vi "Load_Rabi_MW_Change.vi"(0 "Numeric 2":i32, 1 "Numeric":i32, 2 "?":bool=TRUE, 3 "MW Step Size":dbl=2e-09) -> (7 "MW":dbl)   [LabVIEW 2024]
uses:
  <vilib>/Utility/error.llb/DialogTypeEnum.ctl
  SpinCore_API_file_location.vi
panel:
  out "x+y 3":dbl
  out "output array 2":T1(array[cluster])
  out "x+y 2":dbl
  out "output array":T1(array[cluster])
  in  "Instructions":T1(array[cluster])=[{"Instruct Data"=0, "Op Code"=0, "Flags"=[FALSE, FALSE, TRUE, FALSE, FALSE, FALSE, FALSE, TRUE, FALSE, FALSE, FALSE, FALSE, FALSE, FALSE, FALSE, FALSE, FALSE, FALSE, FALSE, FALSE, FALSE, FALSE, FALSE, TRUE], "Comments"="0 Dark", "Time (s)"=6e-06}, {"Instruct Data"=0, "Op Code"=0, "Flags"=[TRUE, FALSE, FALSE, FALSE, TRUE, FALSE, FALSE, TRUE, FALSE, FALSE, FALSE, FALSE, FALSE, FALSE, FALSE, FALSE, FALSE, FALSE, FALSE, FALSE, FALSE, FALSE, FALSE, FALSE], "Comments"="1 PI", "Time (s)"=1e-08}, {"Instruct Data"=0, "Op Code"=0, "Flags"=[FALSE, TRUE, FALSE, FALSE, FALSE, FALSE, FALSE, TRUE, FALSE, FALSE, FALSE, FALSE, FALSE, FALSE, FALSE, FALSE, FALSE, FALSE, FALSE, FALSE, FALSE, FALSE, FALSE, FALSE], "Comments"="2 AOM Delay", "Time (s)"=5e-07}, {"Instruct Data"=0, "Op Code"=0, "Flags"=[FALSE, TRUE, FALSE, FALSE, FALSE, FALSE, FALSE, FALSE, FALSE, FALSE, FALSE, FALSE, FALSE, FALSE, FALSE, FALSE, FALSE, FALSE, FALSE, FALSE, FALSE, FALSE, FALSE, FALSE], "Comments"="3 AOM inhibit off", "Time (s)"=5e-07}, {"Instruct Data"=0, "Op Code"=0, "Flags"=[FALSE, TRUE, FALSE, FALSE, FALSE, FALSE, FALSE, TRUE, FALSE, FALSE, FALSE, FALSE, FALSE, FALSE, FALSE, FALSE, FALSE, FALSE, FALSE, FALSE, FALSE, FALSE, FALSE, FALSE], "Comments"="4 AOM", "Time (s)"=5e-06}, {"Instruct Data"=0, "Op Code"=0, "Flags"=[FALSE, FALSE, FALSE, FALSE, FALSE, FALSE, FALSE, TRUE, FALSE, FALSE, FALSE, FALSE, FALSE, FALSE, FALSE, FALSE, FALSE, FALSE, FALSE, FALSE, FALSE, FALSE, FALSE, FALSE], "Comments"="5 Dark", "Time (s)"=6e-06}, {"Instruct Data"=0, "Op Code"=0, "Flags"=[FALSE, TRUE, FALSE, FALSE, FALSE, FALSE, FALSE, TRUE, FALSE, FALSE, FALSE, FALSE, FALSE, FALSE, FALSE, FALSE, FALSE, FALSE, FALSE, FALSE, FALSE, FALSE, FALSE, FALSE], "Comments"="6 AOM delay", "Time (s)"=5e-07}, {"Instruct Data"=0, "Op Code"=0, "Flags"=[FALSE, TRUE, FALSE, FALSE, FALSE, FALSE, FALSE, FALSE, FALSE, FALSE, FALSE, FALSE, FALSE, FALSE, FALSE, FALSE, FALSE, FALSE, FALSE, FALSE, FALSE, FALSE, FALSE, FALSE], "Comments"="7 AOM inhibit", "Time (s)"=5e-07}, {"Instruct Data"=0, "Op Code"=6, "Flags"=[FALSE, TRUE, FALSE, FALSE, FALSE, FALSE, FALSE, TRUE, FALSE, FALSE, FALSE, FALSE, FALSE, FALSE, FALSE, FALSE, FALSE, FALSE, FALSE, FALSE, FALSE, FALSE, FALSE, FALSE], "Comments"="8 AOM", "Time (s)"=5e-06}, {"Instruct Data"=0, "Op Code"=0, "Flags"=[FALSE, TRUE, FALSE, FALSE, FALSE, FALSE, FALSE, FALSE, FALSE, FALSE, FALSE, FALSE, FALSE, FALSE, FALSE, FALSE, FALSE, FALSE, FALSE, FALSE, FALSE, FALSE, FALSE, FALSE], "Comments"="9", "Time (s)"=2e-06}, {"Instruct Data"=0, "Op Code"=0, "Flags"=[FALSE, TRUE, TRUE, FALSE, FALSE, FALSE, FALSE, FALSE, FALSE, FALSE, FALSE, FALSE, FALSE, FALSE, FALSE, FALSE, FALSE, FALSE, FALSE, FALSE, FALSE, FALSE, FALSE, FALSE], "Comments"="10", "Time (s)"=1e-07}, {"Instruct Data"=0, "Op Code"=0, "Flags"=[FALSE, TRUE, FALSE, FALSE, FALSE, FALSE, FALSE, FALSE, FALSE, FALSE, FALSE, FALSE, FALSE, FALSE, FALSE, FALSE, FALSE, FALSE, FALSE, FALSE, FALSE, FALSE, FALSE, FALSE], "Comments"="11", "Time (s)"=2.9e-06}, {"Instruct Data"=0, "Op Code"=6, "Flags"=[FALSE, FALSE, FALSE, FALSE, FALSE, FALSE, FALSE, FALSE, FALSE, FALSE, FALSE, FALSE, FALSE, FALSE, FALSE, FALSE, FALSE, FALSE, FALSE, FALSE, FALSE, FALSE, FALSE, FALSE], "Comments"="12", "Time (s)"=1e-06}] {"Time (s)" format="%.3p"; "Op Code" items=["Continue", "Stop", "Loop", "End Loop", "JSR", "RTS", "Branch", "Long Delay", "Wait"]}
  in  "# of Instructions":u32=9
  in  "clock_freq (MHz)":dbl=500.0
  # "1) MW indicator\n2) AOM\n3) DAQ\n4) I\n5)Q\n8) Inhibit\n24) Start_Trig"
  # "1"
  # "2"
  # "3"
  # "4"
  # "5"
  # "6"
  # "7"
  # "8"
  # "9"
  # "10"
  # "11"
  # "12"
  # "13"
  # "14"
  # "15"
  # "16"
  # "17"
  # "18"
  # "19"
  # "20"
  # "21"
  # "22"
  # "23"
  # "24"
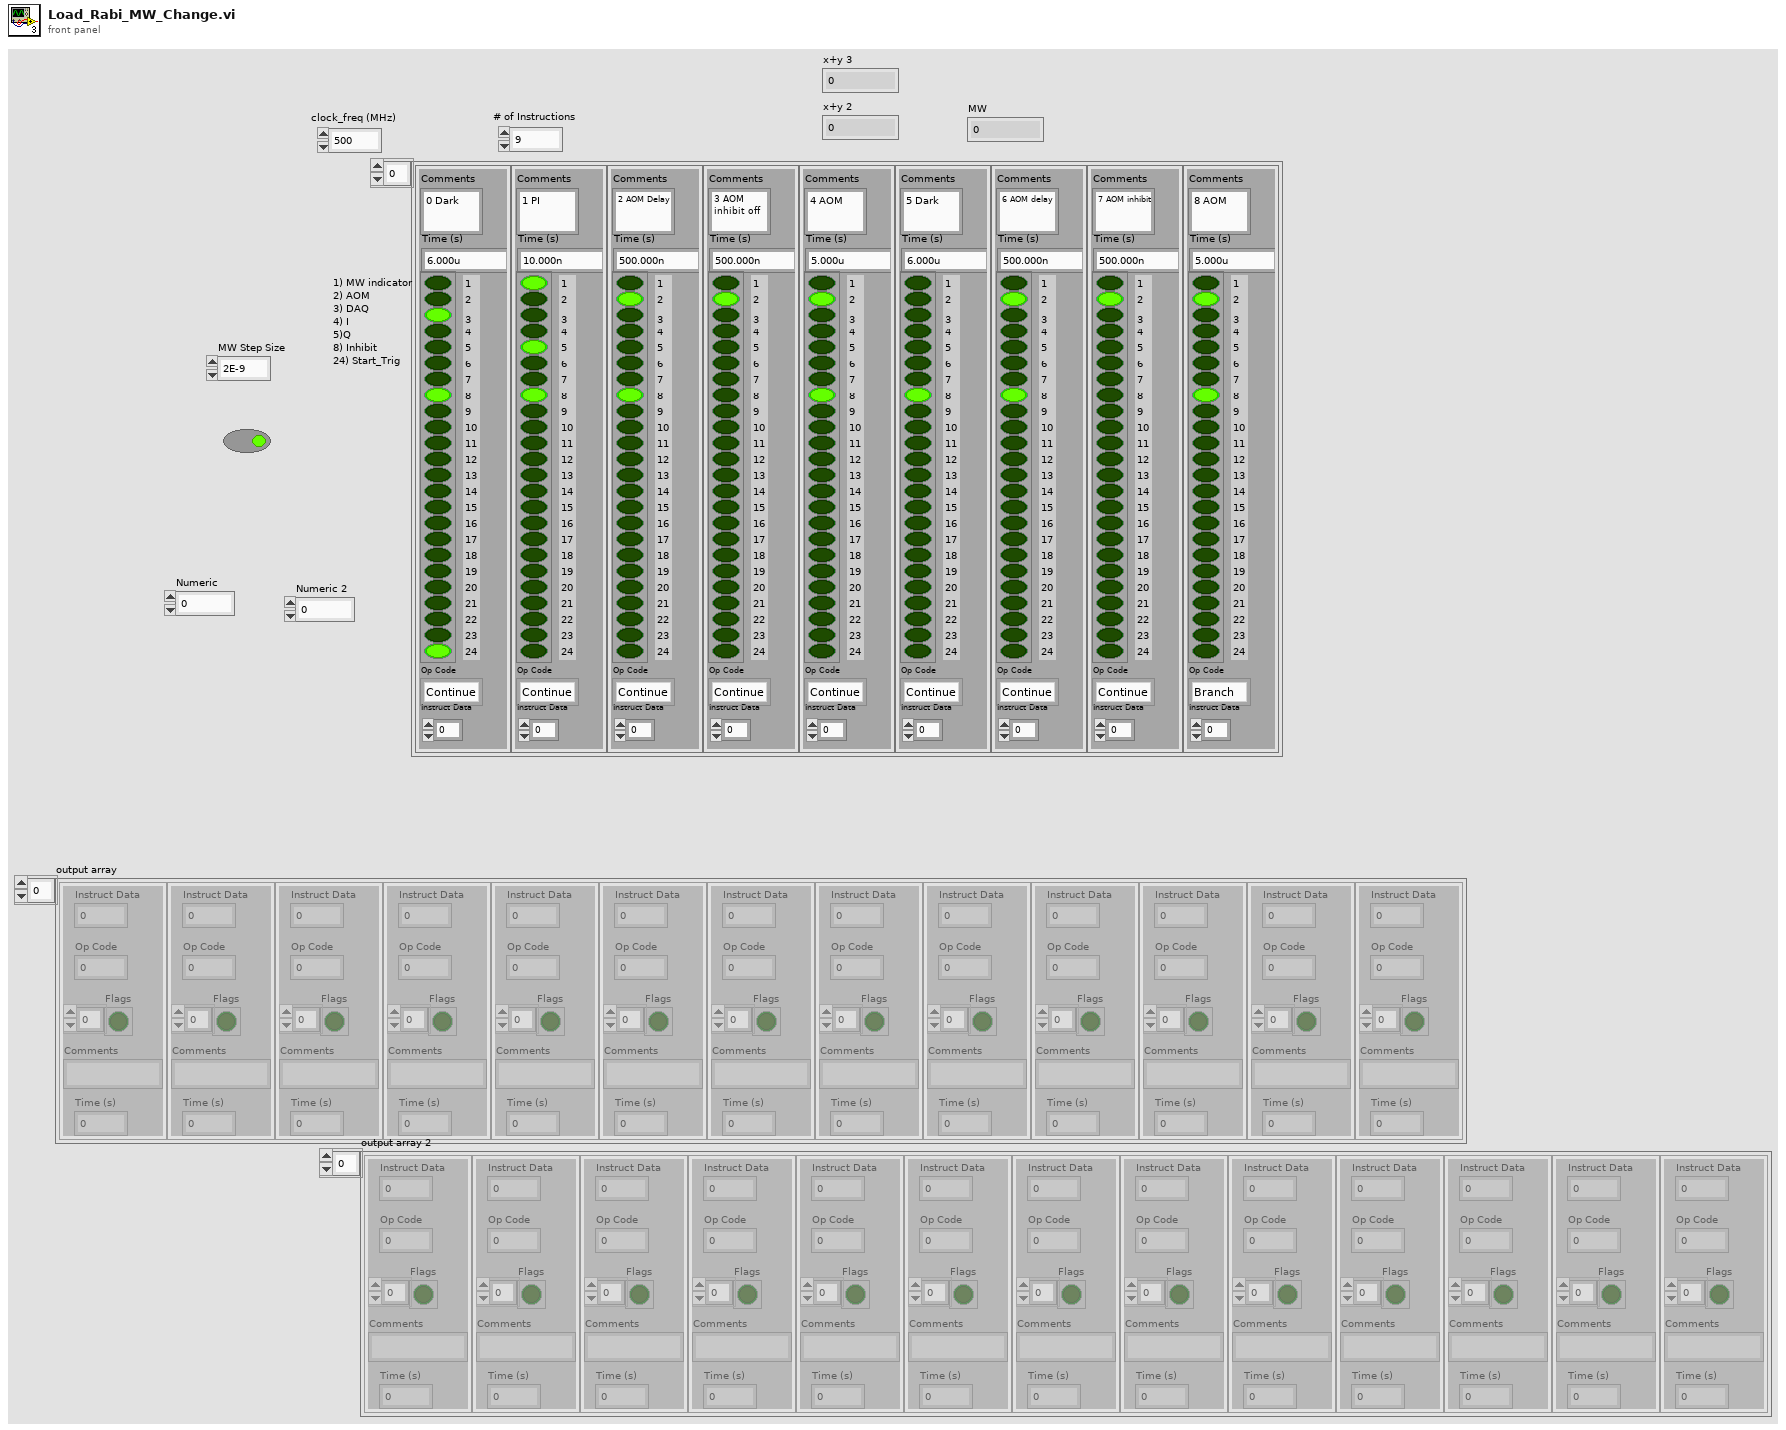
[diagram p1: front panel]
types:
  T1 = cluster{"Instruct Data":i32, "Op Code":i32, "Flags":bool[], "Comments":string, "Time (s)":dbl}[]
  T2 = typedef "DialogTypeEnum.ctl" = enum16{"no dialog", "OK message", "continue or stop message", "auto error handling dialog", "OK message + warnings", "continue/stop + warnings"}
  T3 = enum16{"Pulse Program", "Frequency Registers", "TX Phase Registers", "RX Phase Registers"}
  T4 = cluster{"Instruct Data":i32, "Op Code":i32, "Flags":bool[], "Comments":string, "Time (s)":dbl}
  T5 = cluster{"Instruct Data":i32, "Op Code":i32, "Flags":bool[], "Comments":string, dbl}
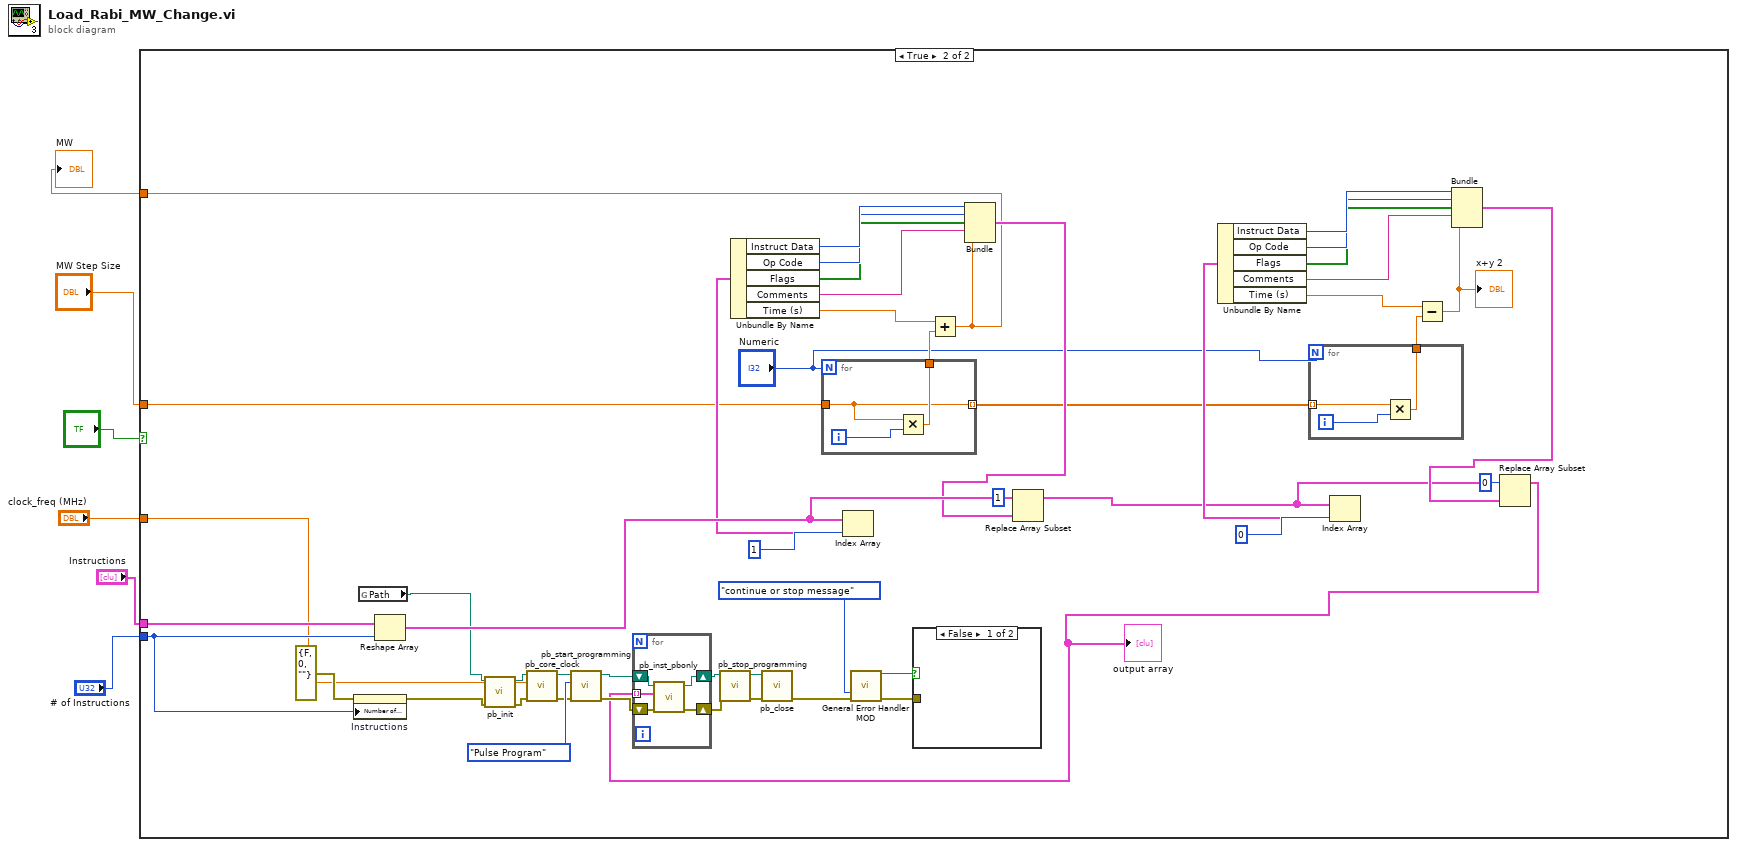
[diagram p0: block diagram]
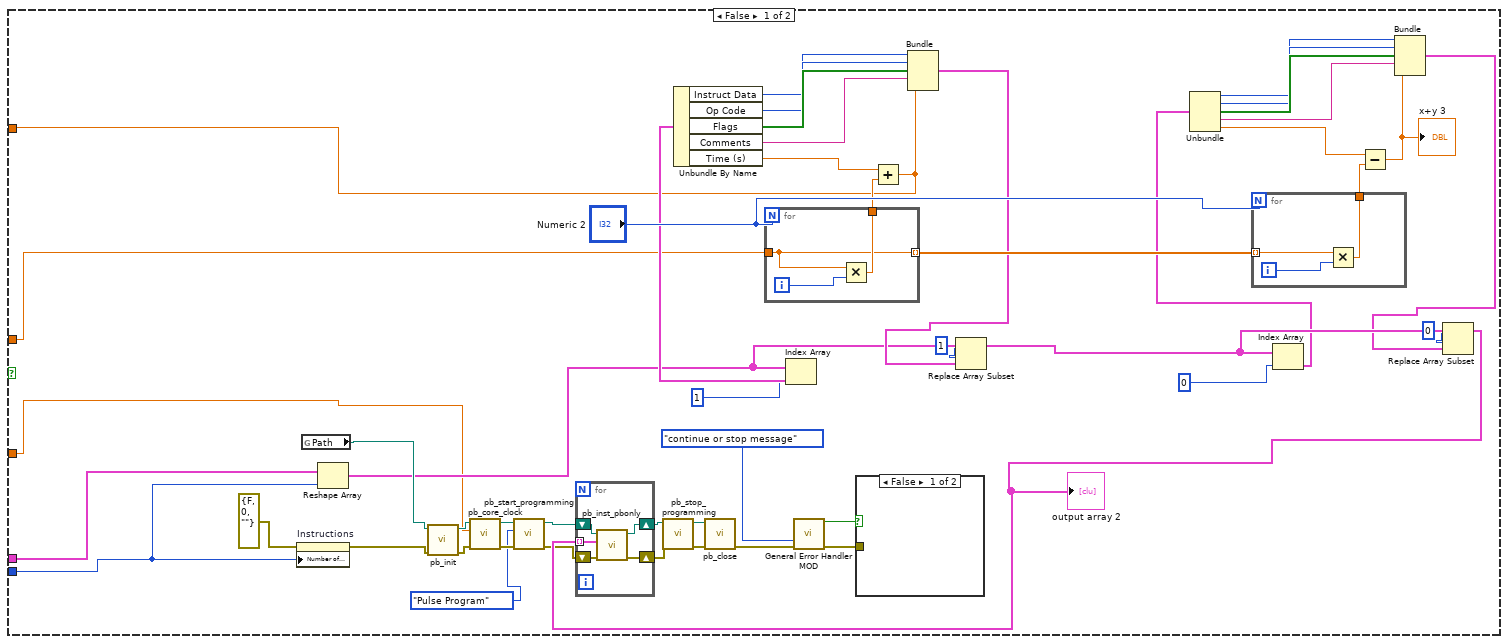
[diagram p2: hidden frame]
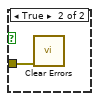
[diagram p3: hidden frame]
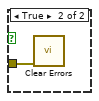
[diagram p4: hidden frame]
diagram:
  n1 = case shown="True" "?" {
    tunnel: "Instructions" -> [w11 w72]
    tunnel: "# of Instructions" -> [w10 w71]
    tunnel: "clock_freq (MHz)" -> [w12 w70]
    tunnel: "MW Step Size" -> [w9 w69]
    tunnel: [w8 w68] -> w1
    frame False {
      n2 = property on="Instructions" class="Arr (strict)"(error in=errorcluster {"status"=FALSE, "code"=0, "source"=""} ("error in (no error)"), "Number of Columns"=w10) -> (error out=w41:errorcluster)  [unwired: 1 in, 1 out]
      n3 = global read "SpinCore_API_file_location.vi" "Path"() -> (w40:path)
      n4 = Reshape Array "Reshape Array"(w11, w10) -> (w36:T1)
      n5 = call "pb_init.vi"("error in (no error)"=w41, "path in"=w40) -> ("error out"=w42:errorcluster, "path out"=w43:path)  [unwired: 8 in]
      n6 = call "pb_core_clock.vi"("error in (no error)"=w42, "clock_freq (MHz)"=w12, "path in"=w43) -> ("error out"=w29:errorcluster, "path out"=w28:path)  [unwired: 7 in]
      n7 = call "pb_start_programming.vi"("error in (no error)"=w29, "Device"=T3."Pulse Program", "path in"=w28) -> ("error out"=w23:errorcluster, "path out"=w20:path)  [unwired: 1 in, 6 out]
      n8 = for {
        N: "Numeric 2" -> [_]
        tunnel: [w60] -> w39
        tunnel: [w59] -> w55 mode=indexing
        tunnel: w9 -> [w59]
        i -> [w61]
        n9 = Multiply(x=w59, y=w61) -> (x*y=w60:dbl)
      }
      n10 = Index Array "Index Array"(array=w36, index=1) -> (element=w37:T4)
      n11 = Unbundle By Name "Unbundle By Name"(w37) -> ("Instruct Data"=w31:i32, "Op Code"=w32:i32, "Flags"=w33:bool[], "Comments"=w34:string, "Time (s)"=w35:dbl)
      n12 = Add(x=w35, y=w39) -> (x+y=w8:dbl)
      n13 = Bundle("Instruct Data"=w31, "Op Code"=w32, "Flags"=w33, "Comments"=w34, w8) -> (w38:T5)  [unwired: 1 in]
      n14 = Replace Array Subset "Replace Array Subset"(array=w36, new element=w38, index=1) -> (w52:T1)
      n15 = for {
        N: "Numeric 2" -> [_]
        tunnel: [w57] -> w51
        tunnel: w55 -> [w56] mode=indexing
        i -> [w58]
        n16 = Multiply(x=w56, y=w58) -> (x*y=w57:dbl)
      }
      n17 = Index Array "Index Array"(array=w52, index=0) -> (element=w7:T4)
      n18 = Unbundle(w7) -> ("Instruct Data"=w44:i32, "Op Code"=w45:i32, "Flags"=w46:bool[], "Comments"=w47:string, "Time (s)"=w48:dbl)
      n19 = Subtract(x=w48, y=w51) -> (x-y=w49:dbl)
      "x+y 3" <- w49
      n20 = Bundle("Instruct Data"=w44, "Op Code"=w45, "Flags"=w46, "Comments"=w47, w49) -> (w50:T5)  [unwired: 1 in]
      n21 = Replace Array Subset "Replace Array Subset"(array=w52, new element=w50, index=0) -> (w53:T1)
      "output array 2" <- w53
      n22 = for {
        tunnel: w53 -> [w64] mode=indexing
        shift-right: [w66] -> w22
        shift-left: w20 -> [w67]
        shift-right: [w63] -> w24
        shift-left: w23 -> [w65]
        n23 = call "pb_inst_pbonly.vi"("error in (no error)"=w65, "PB Instruction"=w64, "path in"=w67) -> ("error out"=w63:errorcluster, "path out"=w66:path)  [unwired: 2 in, 5 out]
      }
      n24 = call "pb_stop_programming.vi"("error in (no error)"=w24, "path in"=w22) -> ("error out"=w25:errorcluster, "path out"=w21:path)  [unwired: 1 in, 7 out]
      n25 = call "pb_close.vi"("error in (no error)"=w25, "path in"=w21) -> ("error out"=w30:errorcluster)  [unwired: 9 out]
      n26 = call "General Error Handler MOD.vi"("type of dialog (OK msg:1)"=DialogTypeEnum."continue or stop message", "error in (no error)"=w30) -> ("STOP?"=w27:bool, "error out"=w26:errorcluster)  [unwired: 12 out]
      n27 = case shown="False" w27 {
        tunnel: w26 -> [_ w62]
        frame False {
        }
        frame True {
          n28 = call <vilib>:"Clear Errors.vi"("error in (no error)"=w62) -> ()  [unwired: 1 in, 6 out]
        }
      }
    }
    frame True {
      n29 = property on="Instructions" class="Arr (strict)"(error in=errorcluster {"status"=FALSE, "code"=0, "source"=""} ("error in (no error)"), "Number of Columns"=w71) -> (error out=w91:errorcluster)  [unwired: 1 in, 1 out]
      n30 = global read "SpinCore_API_file_location.vi" "Path"() -> (w92:path)
      n31 = Reshape Array "Reshape Array"(w72, w71) -> (w97:T1)
      n32 = call "pb_init.vi"("error in (no error)"=w91, "path in"=w92) -> ("error out"=w90:errorcluster, "path out"=w89:path)  [unwired: 8 in]
      n33 = call "pb_core_clock.vi"("error in (no error)"=w90, "clock_freq (MHz)"=w70, "path in"=w89) -> ("error out"=w105:errorcluster, "path out"=w106:path)  [unwired: 7 in]
      n34 = call "pb_start_programming.vi"("error in (no error)"=w105, "Device"=T3."Pulse Program", "path in"=w106) -> ("error out"=w112:errorcluster, "path out"=w116:path)  [unwired: 1 in, 6 out]
      n35 = for {
        N: "Numeric" -> [_]
        tunnel: [w121] -> w93
        tunnel: [w120] -> w74 mode=indexing
        tunnel: w69 -> [w120]
        i -> [w122]
        n36 = Multiply(x=w120, y=w122) -> (x*y=w121:dbl)
      }
      n37 = Index Array "Index Array"(array=w97, index=1) -> (element=w96:T4)
      n38 = Unbundle By Name "Unbundle By Name"(w96) -> ("Instruct Data"=w102:i32, "Op Code"=w101:i32, "Flags"=w100:bool[], "Comments"=w99:string, "Time (s)"=w98:dbl)
      n39 = Add(x=w98, y=w93) -> (x+y=w68:dbl)
      n40 = Bundle("Instruct Data"=w102, "Op Code"=w101, "Flags"=w100, "Comments"=w99, w68) -> (w94:T5)  [unwired: 1 in]
      n41 = Replace Array Subset "Replace Array Subset"(array=w97, new element=w94, index=1) -> (w77:T1)
      n42 = for {
        N: "Numeric" -> [_]
        tunnel: [w118] -> w78
        tunnel: w74 -> [w117] mode=indexing
        i -> [w119]
        n43 = Multiply(x=w117, y=w119) -> (x*y=w118:dbl)
      }
      n44 = Index Array "Index Array"(array=w77, index=0) -> (element=w81:T4)
      n45 = Unbundle By Name "Unbundle By Name"(w81) -> ("Instruct Data"=w87:i32, "Op Code"=w86:i32, "Flags"=w85:bool[], "Comments"=w84:string, "Time (s)"=w83:dbl)
      n46 = Subtract(x=w83, y=w78) -> (x-y=w82:dbl)
      "x+y 2" <- w82
      n47 = Bundle("Instruct Data"=w87, "Op Code"=w86, "Flags"=w85, "Comments"=w84, w82) -> (w79:T5)  [unwired: 1 in]
      n48 = Replace Array Subset "Replace Array Subset"(array=w77, new element=w79, index=0) -> (w76:T1)
      "output array" <- w76
      n49 = for {
        tunnel: w76 -> [w125] mode=indexing
        shift-right: [w127] -> w114
        shift-left: w116 -> [w128]
        shift-right: [w124] -> w111
        shift-left: w112 -> [w126]
        n50 = call "pb_inst_pbonly.vi"("error in (no error)"=w126, "PB Instruction"=w125, "path in"=w128) -> ("error out"=w124:errorcluster, "path out"=w127:path)  [unwired: 2 in, 5 out]
      }
      n51 = call "pb_stop_programming.vi"("error in (no error)"=w111, "path in"=w114) -> ("error out"=w110:errorcluster, "path out"=w115:path)  [unwired: 1 in, 7 out]
      n52 = call "pb_close.vi"("error in (no error)"=w110, "path in"=w115) -> ("error out"=w104:errorcluster)  [unwired: 9 out]
      n53 = call "General Error Handler MOD.vi"("type of dialog (OK msg:1)"=DialogTypeEnum."continue or stop message", "error in (no error)"=w104) -> ("STOP?"=w107:bool, "error out"=w108:errorcluster)  [unwired: 12 out]
      n54 = case shown="False" w107 {
        tunnel: w108 -> [_ w123]
        frame False {
        }
        frame True {
          n55 = call <vilib>:"Clear Errors.vi"("error in (no error)"=w123) -> ()  [unwired: 1 in, 6 out]
        }
      }
    }
  }
  "MW" <- w1
